vi "topology_config.vi"() -> ()   [LabVIEW 2026]
uses:
  <vilib>/addons/_JKI.lib/Serialization/JSON/JKI JSON Serialization.lvlib
panel:
  in  "?":bool
  out "Preview":string
  in  "Clear / Reset":bool
  in  "Generate JSON":bool
  out "Status Message":string
  in  "Save Path":path
  in  "Setting Tab":enum32{"Main", "Advanced"}(tab)
  in  "Nodes Tab":T1(tab)
  in  "PV Array":T2(array[cluster])
  in  "WT Array":T3(array[cluster])
  in  "Gen Array":T4(array[cluster])
  in  "DESD Array":T5(array[cluster])
  in  "Load Array":T6(array[cluster])
  in  "Grid Array":T7(array[cluster])
  in  "Feeders":T8(array[cluster])
  in  "Device ID":cluster{"device_id":string}
  in  "Advanced":T9={"tail_duration_seconds"=86400, "samples_per_day"=1440, "hourly_steps_per_day"=24, "power_signal_prefix"="Power_", "mat_format"="simscape_power_scope"}
  # "Actions"
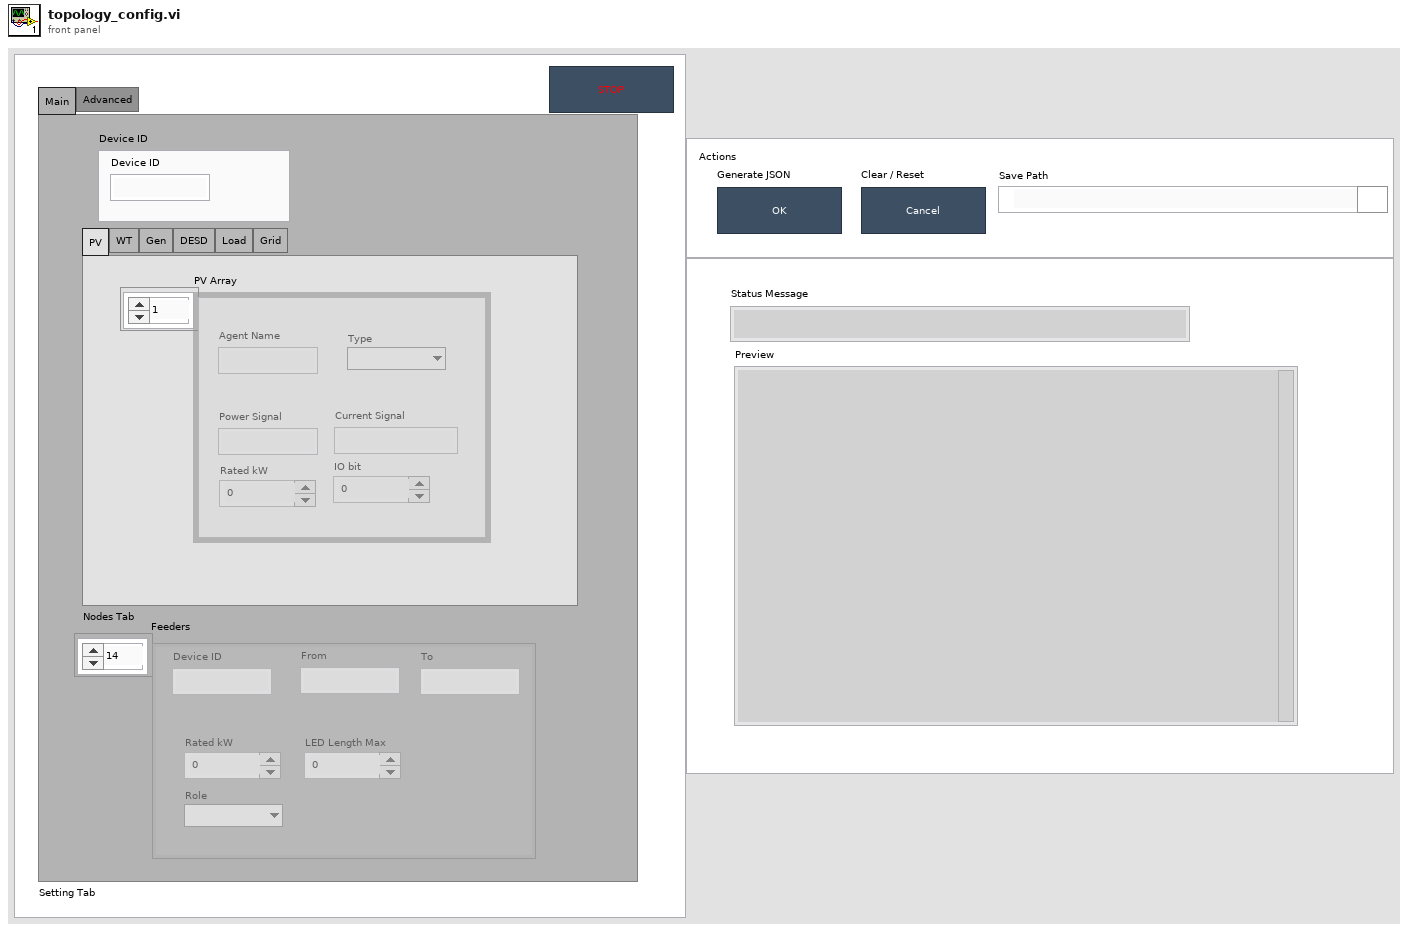
[diagram p1: front panel]
types:
  T1 = enum32{"PV", "WT", "Gen", "DESD", "Load", "Grid"}
  T2 = cluster{"agent_name":string, "power_signal":string, "current_signal":string, "rated_kw":i32, "io_bit":i32, "type 3":enum16{"", "PV", "WT", "Gen", "DESD", "Load", "Grid"}}[]
  T3 = cluster{"agent_name":string, "device_id":string, "power_signal":string, "rated_kw":i32, "io_bit":i32, "type":enum16{"", "PV", "WT", "Gen", "DESD", "Load", "Grid"}, "current_signal":string, "rated_wind_speed_ms":dbl}[]
  T4 = cluster{"agent_name":string, "power_signal":string, "current_signal":string, "rated_kw":i32, "io_bit":i32, "type":enum16{"", "PV", "WT", "Gen", "DESD", "Load", "Grid"}}[]
  T5 = cluster{"agent_name":string, "device_id":string, "power_signal":string, "soc_signal":string, "voltage_signal":string, "current_signal":string, "rated_kw":i32, "io_bit":i32, "capacity_kwh":i32, "type":enum16{"", "PV", "WT", "Gen", "DESD", "Load", "Grid"}}[]
  T6 = cluster{"agent_name":string, "power_signal":string, "current_signal":string, "rated_kw":i32, "io_bit":i32, "priority":enum16{"", "P1", "P2", "P3", "P4"}, "load_type":enum16{"", "Hospital", "CommCenter", "ResArea1", "ResArea2"}, "colocated_with_feeder_node":string, "type":enum16{"", "PV", "WT", "Gen", "DESD", "Load", "Grid"}}[]
  T7 = cluster{"rated_kw":i32, "io_bit":i32, "type":enum16{"", "PV", "WT", "Gen", "DESD", "Load", "Grid"}}[]
  T8 = cluster{"from":string, "to":string, "rated_kw":i32, "led_length_max":i32, "role":enum16{"", "backbone", "main_grid_tie"}, "device_id":string}[]
  T9 = cluster{"tail_duration_seconds":i32, "samples_per_day":i32, "hourly_steps_per_day":i32, "power_signal_prefix":string, "mat_format":string}
  T10 = enum16{"", "Hospital", "CommCenter", "ResArea1", "ResArea2"}
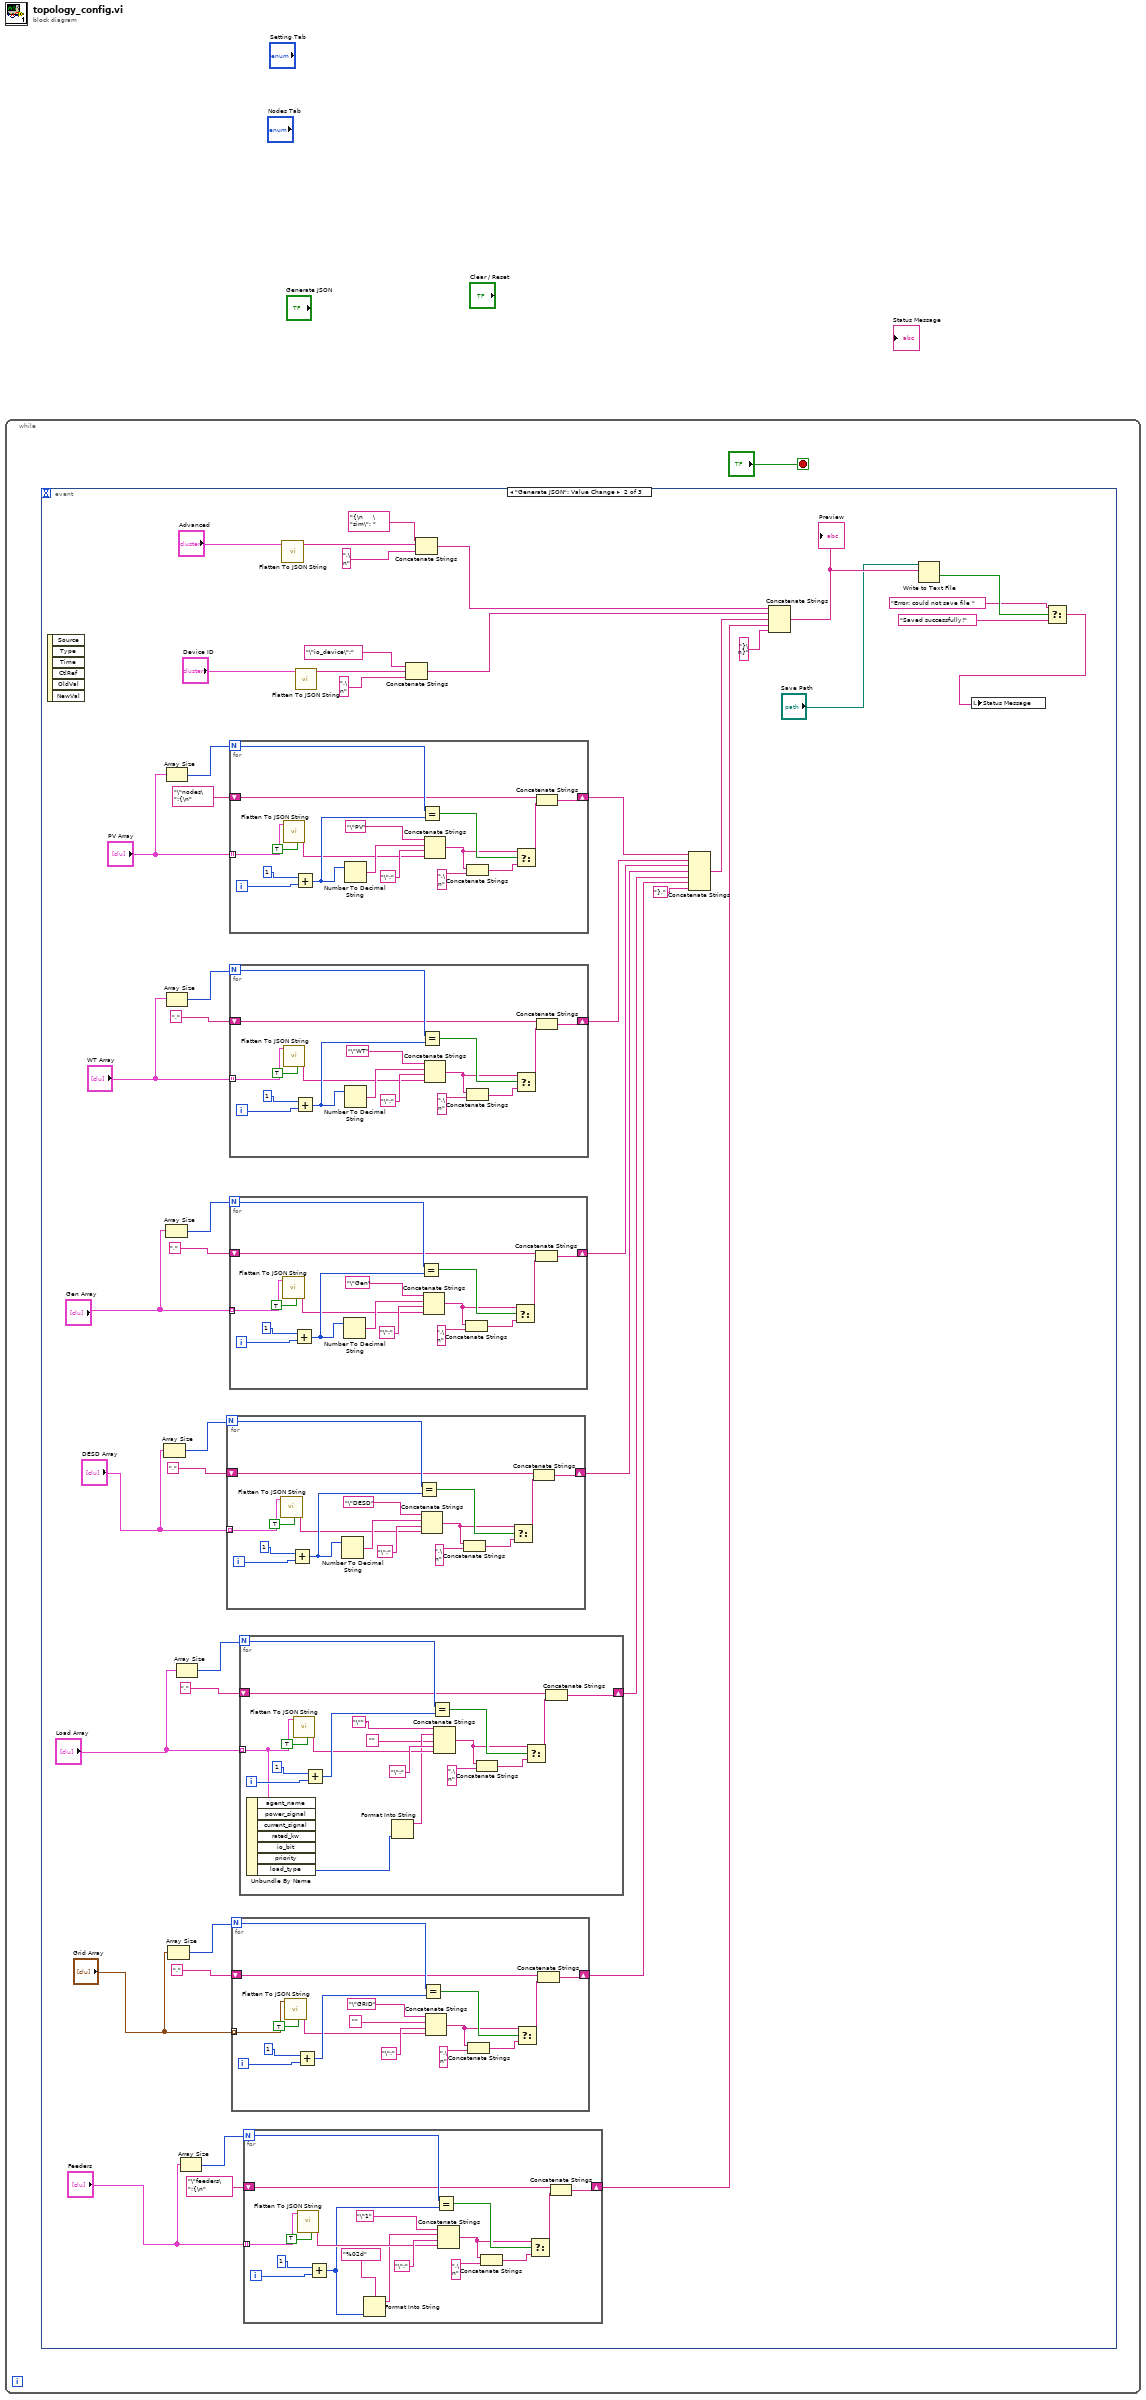
[diagram p0: block diagram]
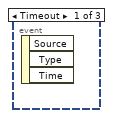
[diagram p2: hidden frame]
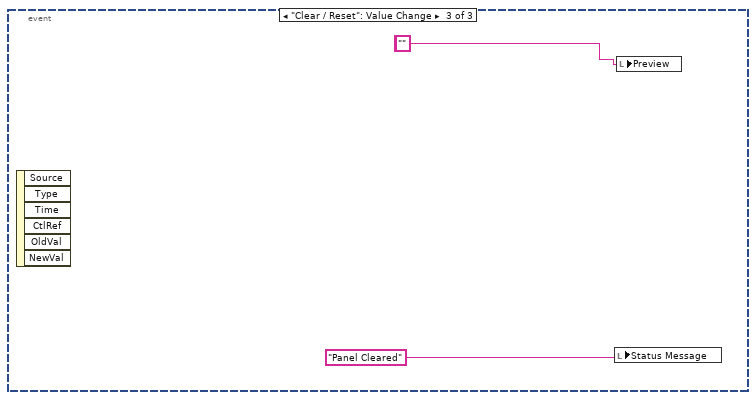
[diagram p3: hidden frame]
diagram:
  n1 = while {
    stop <- "?" stop-if-true
    n2 = event shown="[1] \"Generate JSON\": Value Change" {
      selector: _ -> [_ _ _]
      dyn-events: _ -> [_ _ _]
      timeout: _ -> [_ _ _]
      event Timeout {
        n3 = event-data() -> ()  [unwired: 1 in, 3 out]
      }
      event "Generate JSON": Value Change {
        n4 = event-data() -> ()  [unwired: 1 in, 6 out]
        n5 = Array Size(array="DESD Array") -> (size(s)=w26:i32)
        n6 = Array Size(array="Gen Array") -> (size(s)=w30:i32)
        n7 = Array Size(array="PV Array") -> (size(s)=w37:i32)
        n8 = Array Size(array="WT Array") -> (size(s)=w35:i32)
        n9 = Array Size(array="Grid Array") -> (size(s)=w18:i32)
        n10 = Array Size(array="Load Array") -> (size(s)=w24:i32)
        n11 = Array Size(array="Feeders") -> (size(s)=w13:i32)
        n12 = for {
          N: w26 -> [w115]
          tunnel: "DESD Array" -> [w107] mode=indexing
          shift-right: [w108] -> w21
          shift-left: "," -> [w110]
          i -> [w119]
          n13 = call <vilib>:"Flatten To JSON String.vi"("Enums As String (F)"=TRUE, "Variant"=w107) -> ("JSON String"=w104:string)  [unwired: 8 in, 1 out]
          n14 = Add(x=1, y=w119) -> (x+y=w116:i32)
          n15 = Number To Decimal String(number=w116) -> (decimal integer string=w106:string)  [unwired: 1 in]
          n16 = Equal?(x=w115, y=w116) -> (x = y?=w113:bool)
          n17 = Concatenate Strings("\"DESD", w106, "\":", w104) -> (w112:string)
          n18 = Concatenate Strings(w112, ",\n") -> (w111:string)
          n19 = Select(t=w112, s=w113, f=w111) -> (s? t:f=w109:string)
          n20 = Concatenate Strings(w110, w109) -> (w108:string)
        }
        n21 = for {
          N: w30 -> [w132]
          tunnel: "Gen Array" -> [w124] mode=indexing
          shift-right: [w125] -> w27
          shift-left: "," -> [w127]
          i -> [w136]
          n22 = call <vilib>:"Flatten To JSON String.vi"("Enums As String (F)"=TRUE, "Variant"=w124) -> ("JSON String"=w121:string)  [unwired: 8 in, 1 out]
          n23 = Add(x=1, y=w136) -> (x+y=w133:i32)
          n24 = Number To Decimal String(number=w133) -> (decimal integer string=w123:string)  [unwired: 1 in]
          n25 = Equal?(x=w132, y=w133) -> (x = y?=w130:bool)
          n26 = Concatenate Strings("\"Gen", w123, "\":", w121) -> (w129:string)
          n27 = Concatenate Strings(w129, ",\n") -> (w128:string)
          n28 = Select(t=w129, s=w130, f=w128) -> (s? t:f=w126:string)
          n29 = Concatenate Strings(w127, w126) -> (w125:string)
        }
        n30 = for {
          N: w37 -> [w166]
          tunnel: "PV Array" -> [w158] mode=indexing
          shift-right: [w159] -> w32
          shift-left: "\"nodes\":{\n" -> [w161]
          i -> [w170]
          n31 = call <vilib>:"Flatten To JSON String.vi"("Enums As String (F)"=TRUE, "Variant"=w158) -> ("JSON String"=w155:string)  [unwired: 8 in, 1 out]
          n32 = Add(x=1, y=w170) -> (x+y=w167:i32)
          n33 = Number To Decimal String(number=w167) -> (decimal integer string=w157:string)  [unwired: 1 in]
          n34 = Equal?(x=w166, y=w167) -> (x = y?=w164:bool)
          n35 = Concatenate Strings("\"PV", w157, "\":", w155) -> (w163:string)
          n36 = Concatenate Strings(w163, ",\n") -> (w162:string)
          n37 = Select(t=w163, s=w164, f=w162) -> (s? t:f=w160:string)
          n38 = Concatenate Strings(w161, w160) -> (w159:string)
        }
        n39 = for {
          N: w35 -> [w149]
          tunnel: "WT Array" -> [w141] mode=indexing
          shift-right: [w142] -> w31
          shift-left: "," -> [w144]
          i -> [w153]
          n40 = call <vilib>:"Flatten To JSON String.vi"("Enums As String (F)"=TRUE, "Variant"=w141) -> ("JSON String"=w138:string)  [unwired: 8 in, 1 out]
          n41 = Add(x=1, y=w153) -> (x+y=w150:i32)
          n42 = Number To Decimal String(number=w150) -> (decimal integer string=w140:string)  [unwired: 1 in]
          n43 = Equal?(x=w149, y=w150) -> (x = y?=w147:bool)
          n44 = Concatenate Strings("\"WT", w140, "\":", w138) -> (w146:string)
          n45 = Concatenate Strings(w146, ",\n") -> (w145:string)
          n46 = Select(t=w146, s=w147, f=w145) -> (s? t:f=w143:string)
          n47 = Concatenate Strings(w144, w143) -> (w142:string)
        }
        n48 = for {
          N: w18 -> [w79]
          tunnel: "Grid Array" -> [w71] mode=indexing
          shift-right: [w72] -> w15
          shift-left: "," -> [w74]
          i -> [w83]
          n49 = call <vilib>:"Flatten To JSON String.vi"("Enums As String (F)"=TRUE, "Variant"=w71) -> ("JSON String"=w69:string)  [unwired: 8 in, 1 out]
          n50 = Add(x=1, y=w83) -> (x+y=w80:i32)
          n51 = Equal?(x=w79, y=w80) -> (x = y?=w77:bool)
          n52 = Concatenate Strings("\"GRID", "", "\":", w69) -> (w76:string)
          n53 = Concatenate Strings(w76, ",\n") -> (w75:string)
          n54 = Select(t=w76, s=w77, f=w75) -> (s? t:f=w73:string)
          n55 = Concatenate Strings(w74, w73) -> (w72:string)
        }
        n56 = for {
          N: w24 -> [w99]
          tunnel: "Load Array" -> [w88] mode=indexing
          shift-right: [w92] -> w20
          shift-left: "," -> [w94]
          i -> [w102]
          n57 = Unbundle By Name(w88) -> ("load_type"=w87:T10)  [unwired: 6 out]
          n58 = call <vilib>:"Flatten To JSON String.vi"("Enums As String (F)"=TRUE, "Variant"=w88) -> ("JSON String"=w90:string)  [unwired: 8 in, 1 out]
          n59 = Add(x=1, y=w102) -> (x+y=w100:i32)
          n60 = Format Into String(w87) -> (resulting string=w85:string)  [unwired: 3 in, 1 out]
          n61 = Equal?(x=w99, y=w100) -> (x = y?=w97:bool)
          n62 = Concatenate Strings("\"", w85, "", "\":", w90) -> (w96:string)
          n63 = Concatenate Strings(w96, ",\n") -> (w95:string)
          n64 = Select(t=w96, s=w97, f=w95) -> (s? t:f=w93:string)
          n65 = Concatenate Strings(w94, w93) -> (w92:string)
        }
        n66 = for {
          N: w13 -> [w63]
          tunnel: "Feeders" -> [w55] mode=indexing
          shift-right: [w56] -> w9
          shift-left: "\"feeders\":{\n" -> [w58]
          i -> [w66]
          n67 = call <vilib>:"Flatten To JSON String.vi"("Enums As String (F)"=TRUE, "Variant"=w55) -> ("JSON String"=w53:string)  [unwired: 8 in, 1 out]
          n68 = Add(x=1, y=w66) -> (x+y=w50:i32)
          n69 = Format Into String(format string="%02d", w50) -> (resulting string=w49:string)  [unwired: 2 in, 1 out]
          n70 = Equal?(x=w63, y=w50) -> (x = y?=w61:bool)
          n71 = Concatenate Strings("\"1", w49, "\":", w53) -> (w60:string)
          n72 = Concatenate Strings(w60, ",\n") -> (w59:string)
          n73 = Select(t=w60, s=w61, f=w59) -> (s? t:f=w57:string)
          n74 = Concatenate Strings(w58, w57) -> (w56:string)
        }
        n75 = call <vilib>:"Flatten To JSON String.vi"("Variant"="Advanced") -> ("JSON String"=w46:string)  [unwired: 9 in, 1 out]
        n76 = call <vilib>:"Flatten To JSON String.vi"("Variant"="Device ID") -> ("JSON String"=w44:string)  [unwired: 9 in, 1 out]
        n77 = Concatenate Strings("\"io_device\":", w44, ",\n") -> (w40:string)
        n78 = Concatenate Strings("{\n     \"sim\": ", w46, ",\n") -> (w41:string)
        n79 = Concatenate Strings(w32, w31, w27, w21, w20, w15, "},") -> (w10:string)
        n80 = Concatenate Strings(w41, w40, w10, w9, "}\n}") -> (w4:string)
        "Preview" <- w4
        n81 = Write to Text File(file (use dialog)="Save Path", text=w4) -> (cancelled=w7:bool)  [unwired: 2 in, 2 out]
        n82 = Select(t="Error: could not save file ", s=w7, f="Saved successfully!") -> (s? t:f=w2:string)
        n83 = local write "Status Message"(w2) -> ()
      }
      event "Clear / Reset": Value Change {
        (unwired) ""
        n84 = event-data() -> ()  [unwired: 1 in, 6 out]
        n85 = local write "Status Message"("Panel Cleared") -> ()
        n86 = local write "Preview"("") -> ()
      }
    }
  }
